vi "Get XML.vi"(8 "error in":errorcluster, 11 "ToastBuilder in":refnum<class "ToastBuilder.lvclass">) -> (0 "error out":errorcluster, 2 "GetContent":string, 3 "ToastBuilder out":refnum<class "ToastBuilder.lvclass">)   [LabVIEW 2026, in "ToastNotification.lvlib" / "ToastBuilder.lvclass"]
doc: "ToastSource XML export override for ToastBuilder. Serialize the current native builder content without displaying a notification. Skipped on incoming error. Return the same builder and release the temporary content reference after serialization. GetContent is the resulting XML string, not an acquired .NET reference."
uses:
  ToastBuilder.lvclass
  ToastBuilder.lvclass/ToastBuilder.ctl
  Read Builder Reference.vi
  Write Builder Reference.vi
  Toast Native/Toast Native.lvlib
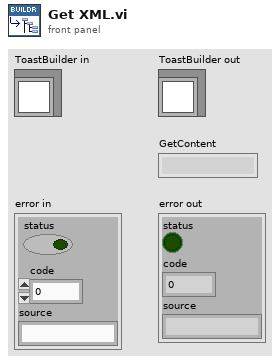
[diagram p1: front panel]
types:
  T1 = typedef "ToastNotification.lvlib/ToastBuilder.lvclass/Builder Reference.ctl" = refnum<k24>
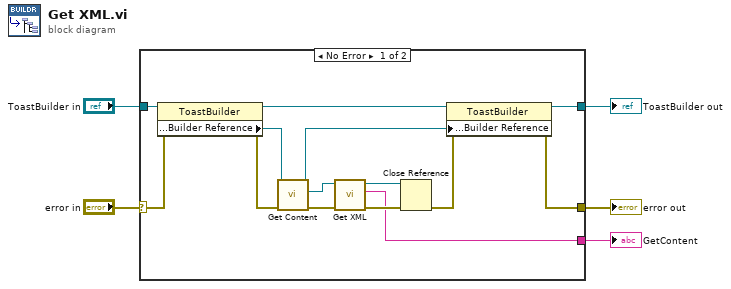
[diagram p0: block diagram]
diagram:
  n1 = case shown="No Error" "error in" {
    selector: "error in" -> [w17 w20]
    tunnel: "ToastBuilder in" -> [w19 w21]
    tunnel: [w16 w21] -> w3
    tunnel: [w15 w20] -> w2
    tunnel: [w6 _] -> w1
    frame No Error {
      n2 = property class="ToastBuilder"(reference=w19, error in=w17) -> (reference out=w18:refnum<class "ToastBuilder.lvclass">, error out=w12:errorcluster, "Public:Properties:Builder Reference"=w14:T1)
      n3 = call "Get Content.vi"("error in (no error)"=w12, "reference"=w14) -> ("error out"=w11:errorcluster, "Content"=w10:refnum<k24>, "reference out"=w13:refnum<k24>)  [unwired: 7 in]
      n4 = call "Get XML.vi"("error in (no error)"=w11, "reference"=w10) -> ("error out"=w8:errorcluster, "GetContent"=w6:string, "reference out"=w9:refnum<k24>)  [unwired: 7 in]
      n5 = Close Reference(reference=w9, error in (no error)=w8) -> (error out=w7:errorcluster)
      n6 = property class="ToastBuilder"(reference=w18, error in=w7, "Public:Properties:Builder Reference"=w13) -> (reference out=w16:refnum<class "ToastBuilder.lvclass">, error out=w15:errorcluster)
    }
    frame Error {
    }
  }
  "ToastBuilder out" <- w3
  "error out" <- w2
  "GetContent" <- w1
